vi "Install Package.vi"(8 "error in":errorcluster, 9 "include recommended packages? (F)":bool, 10 "version":string, 11 "package name":string) -> (0 "error out":errorcluster, 2 "installed version":string, 3 "package name out":string)   [LabVIEW 2014, in "NIPM_API.lvlib"]
doc: "Installs the specified package on this computer.\n\nNote: This VI will launch a Windows dialog asking for permission to run and requires the user to have admin rights.\n\nINPUT(s)\n<B>Package name</B>: Specifies the package to install.\n\n<B>Version</B>:\nIf the version input is left unwired and no version of the package is currently installed, this VI will install the latest version of the package available from the registered feeds on the computer.\nIf the version input is left unwired and any version of the package is currently installed, this VI will output an error.\n\nIf the version input is wired and a different version of the package is installed, this VI will upgrade or downgrade the package to the specified version.\nIf the version input is wired and the specified version of the package is already installed, this VI will output an error.\n\n<B>Include recommended packages</B>: Also install all recommended packages of the specified package.\n\nOUTPUT(s)\n<B>Package name</B>: Outputs the requested package to install.\n\n<B>Installed version</B>: Outputs the currently installed version of the specified package after this VI tries to install the package."
uses:
  NIPM_API.lvlib
  _support/Version Comparison Operator.ctl
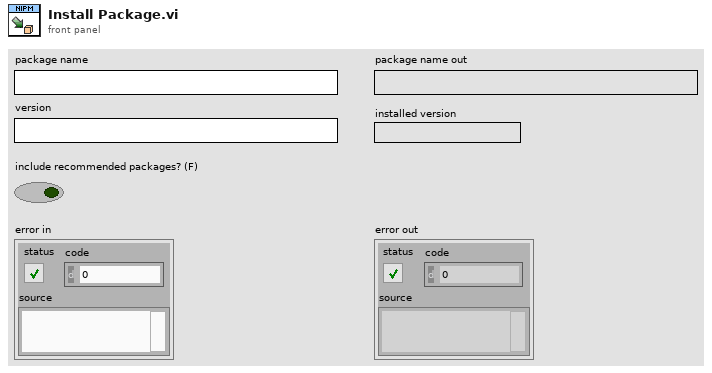
[diagram p1: front panel]
types:
  T1 = typedef "NIPM_API.lvlib/Version Comparison Operator.ctl" = enum16{">", ">=", "=", "!=", "<=", "<"}
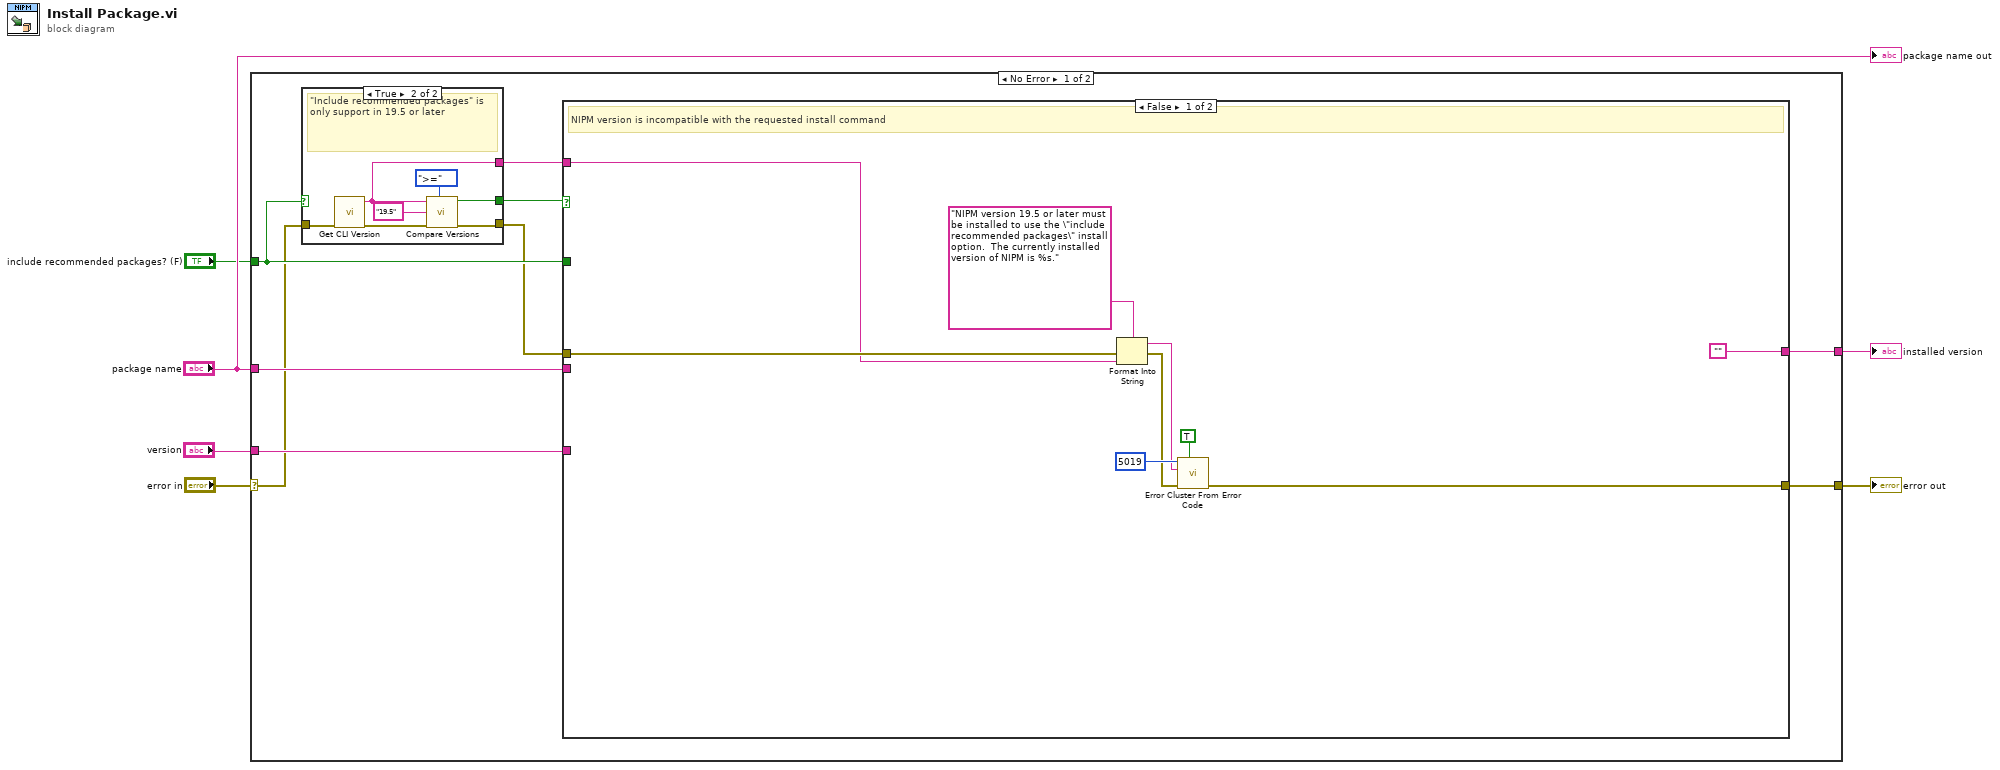
[diagram p0: block diagram]
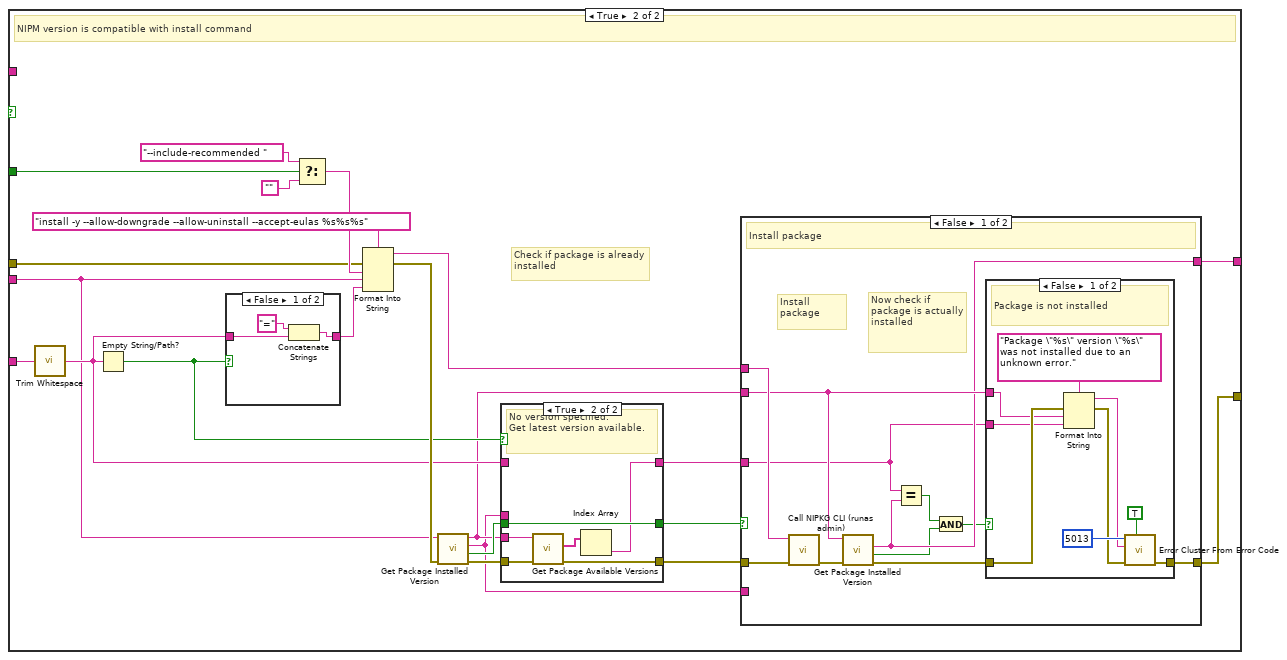
[diagram p2: hidden frame]
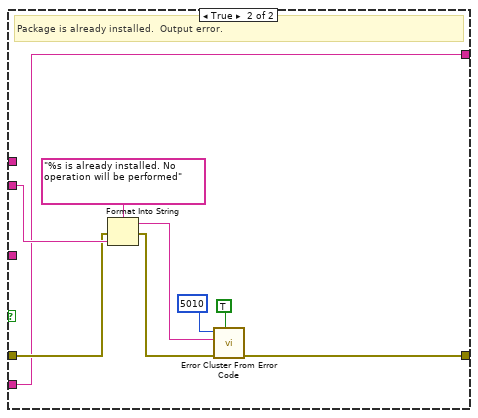
[diagram p4: hidden frame]
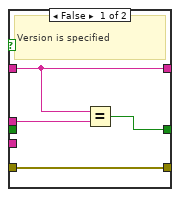
[diagram p5: hidden frame]
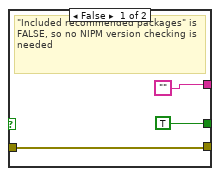
[diagram p7: hidden frame]
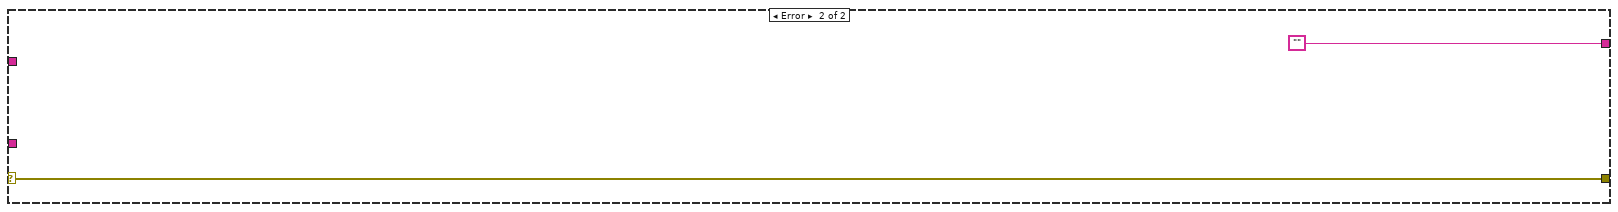
[diagram p8: hidden frame]
diagram:
  n1 = case shown="No Error" "error in" {
    selector: "error in" -> [w10 w102]
    tunnel: [w15 w102] -> w5
    tunnel: "package name" -> [w12 _]
    tunnel: "version" -> [w14 _]
    tunnel: [w13 "" ("standard output")] -> w2
    tunnel: "include recommended packages? (F)" -> [w11 _]
    frame No Error {
      n2 = case shown="True" w11 {
        tunnel: w10 -> [w93 w97]
        tunnel: [w93 w96] -> w9
        tunnel: [TRUE ("Satisfied?") w95] -> w8
        tunnel: ["" w94] -> w7
        frame False {
          # "\"Included recommended packages\" is FALSE, so no NIPM version checking is needed"
        }
        frame True {
          # "\"Include recommended packages\" is only support in 19.5 or later"
          n3 = call "Get CLI Version.vi"("error in"=w97) -> ("error out"=w98:errorcluster, "full version string"=w94:string)  [unwired: 9 in]
          n4 = call "Compare Versions.vi"("operator"=Version_Comparison_Operator.">=", "error in"=w98, "version y"="19.5", "version x"=w94) -> ("error out"=w96:errorcluster, "Satisfied?"=w95:bool)  [unwired: 6 in]
        }
      }
      n5 = case shown="False" w8 {
        tunnel: [w18 w42] -> w15
        tunnel: w14 -> [_ w40]
        tunnel: ["" w38] -> w13
        tunnel: w12 -> [_ w28]
        tunnel: w11 -> [_ w26]
        tunnel: w9 -> [w19 w25]
        tunnel: w7 -> [w16 _]
        frame False {
          # "NIPM version is incompatible with the requested install command"
          n6 = Format Into String(format string="NIPM version 19.5 or later must be installed to use the \"include recommended packages\" install option.  The currently installed version of NIPM is %s.", error in=w19, w16) -> (resulting string=w20:string, error out=w21:errorcluster)  [unwired: 1 in]
          n7 = call <vilib>:"Error Cluster From Error Code.vi"("show call chain? (False)"=TRUE, "error in (no error)"=w21, "error message (\"\")"=w20, "error code (0)"=5019) -> ("error out"=w18:errorcluster)  [unwired: 5 in]
        }
        frame True {
          # "Check if package is already installed"
          # "NIPM version is compatible with install command"
          n8 = call <vilib>:"Trim Whitespace.vi"("string"=w40) -> ("trimmed string"=w39:string)  [unwired: 1 in]
          n9 = Empty String/Path?(string/path=w39) -> (empty?=w41:bool)
          n10 = case shown="False" w41 {
            tunnel: w39 -> [w89 w90]
            tunnel: [w87 w90] -> w45
            frame False {
              n11 = Concatenate Strings("=" ("string"), w89) -> (w87:string)
            }
            frame True {
            }
          }
          n12 = Select(t="--include-recommended ", s=w26, f="") -> (s? t:f=w27:string)
          n13 = Format Into String(format string="install -y --allow-downgrade --allow-uninstall --accept-eulas %s%s%s", error in=w25, w27, w28, w45) -> (resulting string=w43:string, error out=w44:errorcluster)  [unwired: 1 in]
          n14 = call "Get Package Installed Version.vi"("error in"=w44, "package name"=w28) -> ("error out"=w34:errorcluster, "installed?"=w37:bool, "installed version"=w31:string, "package name out"=w32:string)  [unwired: 6 in]
          n15 = case shown="True" w41 {
            tunnel: w37 -> [_ w86]
            tunnel: w31 -> [w80 _]
            tunnel: w39 -> [w78 _]
            tunnel: [w79 w86] -> w36
            tunnel: [w78 w83] -> w35
            tunnel: w34 -> [w77 w85]
            tunnel: [w77 w82] -> w33
            tunnel: w32 -> [_ w81]
            frame False {
              # "Version is specified"
              n16 = Equal?(x=w78, y=w80) -> (x = y?=w79:bool)
            }
            frame True {
              # "No version specified.\nGet latest version available."
              n17 = call "Get Package Available Versions.vi"("error in"=w85, "package name"=w81) -> ("error out"=w82:errorcluster, "versions"=w84:string[])  [unwired: 7 in, 1 out]
              n18 = Index Array(array=w84) -> (element=w83:string)  [unwired: 1 in]
            }
          }
          n19 = case shown="False" w36 {
            tunnel: w43 -> [w57 _]
            tunnel: [w53 w69] -> w42
            tunnel: w33 -> [w56 w71]
            tunnel: w32 -> [w52 w73]
            tunnel: w35 -> [w50 _]
            tunnel: [w51 w68] -> w38
            tunnel: w31 -> [_ w68]
            frame False {
              # "Install package"
              # "Now check if package is actually installed"
              # "Install package"
              n20 = call "Call NIPKG CLI (runas admin).vi"("error in (no error)"=w56, "command"=w57) -> ("error out"=w55:errorcluster)  [unwired: 9 in]
              n21 = call "Get Package Installed Version.vi"("error in"=w55, "package name"=w52) -> ("error out"=w54:errorcluster, "installed?"=w47:bool, "installed version"=w51:string)  [unwired: 6 in, 1 out]
              n22 = Equal?(x=w50, y=w51) -> (x = y?=w49:bool)
              n23 = And(x=w49, y=w47) -> (x .and. y?=w48:bool)
              n24 = case shown="False" w48 {
                tunnel: w54 -> [w61 w67]
                tunnel: [w64 w67] -> w53
                tunnel: w52 -> [w60 _]
                tunnel: w50 -> [w58 _]
                frame False {
                  # "Package is not installed"
                  n25 = Format Into String(format string="Package \"%s\" version \"%s\" was not installed due to an unknown error.", error in=w61, w60, w58) -> (resulting string=w59:string, error out=w62:errorcluster)  [unwired: 1 in]
                  n26 = call <vilib>:"Error Cluster From Error Code.vi"("show call chain? (False)"=TRUE, "error in (no error)"=w62, "error message (\"\")"=w59, "error code (0)"=5013) -> ("error out"=w64:errorcluster)  [unwired: 5 in]
                }
                frame True {
                  # "Package has installed successfully."
                }
              }
            }
            frame True {
              # "Package is already installed.  Output error."
              n27 = Format Into String(format string="%s is already installed. No operation will be performed", error in=w71, w73) -> (resulting string=w72:string, error out=w70:errorcluster)  [unwired: 1 in]
              n28 = call <vilib>:"Error Cluster From Error Code.vi"("show call chain? (False)"=TRUE, "error in (no error)"=w70, "error message (\"\")"=w72, "error code (0)"=5010) -> ("error out"=w69:errorcluster)  [unwired: 5 in]
            }
          }
        }
      }
    }
    frame Error {
    }
  }
  "error out" <- w5
  "installed version" <- w2
  "package name out" <- "package name"
